vi "Unpack and Repack Package.vi"() -> ()   [LabVIEW 2020]
uses:
  source/vi_package_building_extensions.lvlib
panel:
  out "error out":errorcluster
  in  "error in (no error)":errorcluster
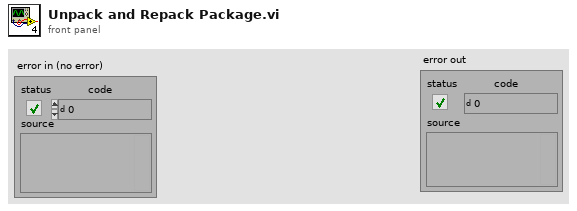
[diagram p1: front panel]
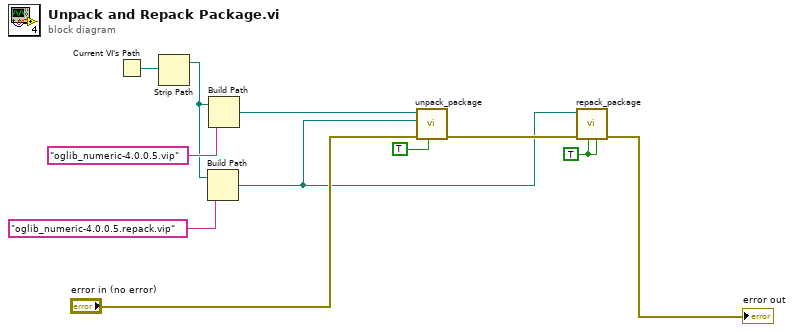
[diagram p0: block diagram]
diagram:
  w2 = TRUE ("Delete Directory to repack (if success)?")
  n1 = Current VI's Path() -> (path=w11:path)
  n2 = Strip Path(path=w11) -> (stripped path=w6:path)  [unwired: 1 out]
  n3 = Build Path(base path=w6, name or relative path="oglib_numeric-4.0.0.5.repack.vip") -> (appended path=w1:path)
  n4 = Build Path(base path=w6, name or relative path="oglib_numeric-4.0.0.5.vip") -> (appended path=w9:path)
  n5 = call "unpack_package.vi"("Overwrite Target Directory if exists (TRUE)?"=TRUE ("Overwrite Target Directory (if exists)?"), "error in (no error)"="error in (no error)", "Target directory (same as Package file if empty)"=w1, "Package File"=w9) -> ("error out"=w5:errorcluster)  [unwired: 5 in, 2 out]
  n6 = call "repack_package.vi"("Delete Directory to repack (TRUE)?"=w2, "Overwrite Target Package File (True)?"=w2, "error in (no error)"=w5, "Package File"=w1) -> ("error out"=→"error out":errorcluster)  [unwired: 7 in]
